vi "Call Get HW Config.vi"(8 "error in":errorcluster, 10 "Refresh Modules":bool, 11 "serverName":string) -> (0 "error out":errorcluster, 3 "HW Config":T1)   [LabVIEW 2020, in "SEECD System Explorer.lvlib"]
uses:
  SEECD System Explorer.lvlib
  Type Defs/Host - HW Config.ctl
  Type Defs/Host - Master.ctl
  Type Defs/Host - Slave.ctl
  Type Defs/IOV Container Contents.ctl
  Type Defs/Host - Module.ctl
  Type Defs/Host - Local Chassis.ctl
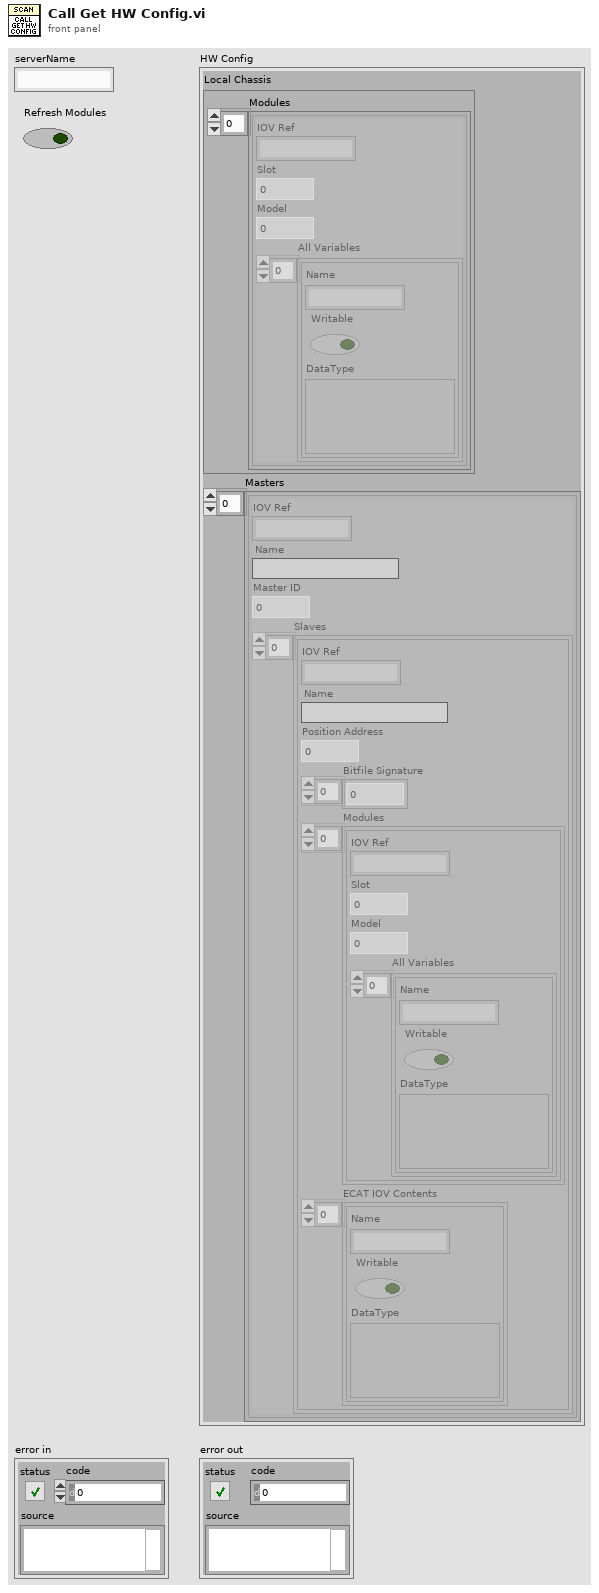
[diagram p1: front panel]
types:
  T1 = typedef "SEECD System Explorer.lvlib/Host - HW Config.ctl" = cluster{"Local Chassis":T2, "Masters":T5[]}
  T2 = typedef "SEECD System Explorer.lvlib/Host - Local Chassis.ctl" = cluster{"Modules":T3[]}
  T3 = typedef "SEECD System Explorer.lvlib/Host - Module.ctl" = cluster{"IOV Ref":string, "Slot":u32, "Model":u32, "All Variables":T4[]}
  T4 = typedef "SEECD System Explorer.lvlib/IOV Container Contents.ctl" = cluster{"Name":string, "Writable":bool, "DataType":variant}
  T5 = typedef "SEECD System Explorer.lvlib/Host - Master.ctl" = cluster{"IOV Ref":string, "Name":string, "Master ID":u32, "Slaves":T6[]}
  T6 = typedef "SEECD System Explorer.lvlib/Host - Slave.ctl" = cluster{"IOV Ref":string, "Name":string, "Position Address":u16, "Bitfile Signature":u8[], "Modules":T3[], "ECAT IOV Contents":T4[]}
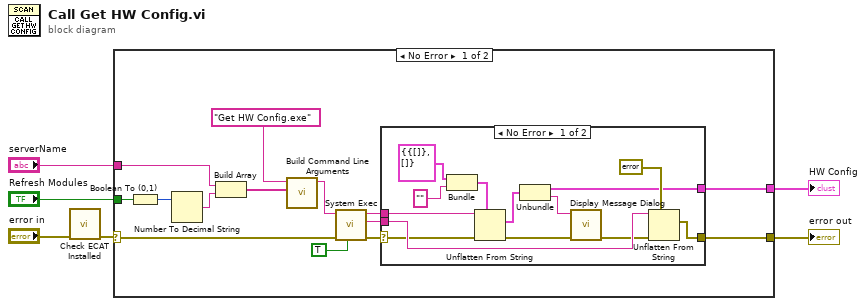
[diagram p0: block diagram]
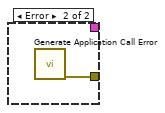
[diagram p2: hidden frame]
diagram:
  n1 = call "Check ECAT Installed.vi"("error in"="error in") -> ("error out"=w1:errorcluster)  [unwired: 10 in]
  n2 = case shown="No Error" w1 {
    selector: w1 -> [w20 w35]
    tunnel: [w7 w35] -> w6
    tunnel: "serverName" -> [w13 _]
    tunnel: [w19 _] -> w3
    tunnel: "Refresh Modules" -> [w10 _]
    frame No Error {
      n3 = Boolean To (0,1)(Boolean=w10) -> (0, 1=w9:i16)
      n4 = Number To Decimal String(number=w9) -> (decimal integer string=w8:string)  [unwired: 1 in]
      n5 = Build Array(w13, w8) -> (w12:string[])
      n6 = call "Build Command Line Arguments.vi"("Arguments"=w12, "Executable File Name"="Get HW Config.exe" ("name or relative path")) -> ("Command Line"=w11:string)  [unwired: 9 in]
      n7 = call <vilib>:"System Exec.vi"("run minimized? (F)"=TRUE, "error in (no error)"=w20, "command line"=w11) -> ("error out"=w18:errorcluster, "standard error"=w16:string, "standard output"=w17:string)  [unwired: 5 in, 1 out]
      n8 = case shown="No Error" w18 {
        selector: w18 -> [w30 _]
        tunnel: [w22 _] -> w19
        tunnel: [w32 w34] -> w7
        tunnel: w17 -> [w29 _]
        tunnel: w16 -> [w31 _]
        frame No Error {
          n9 = Bundle("HW Config"=T1 {"Local Chassis"={"Modules"=[]}, "Masters"=[]}, "") -> (w28:cluster{"HW Config":T1, string})  [unwired: 1 in]
          n10 = Unflatten From String(type=w28, binary string=w29, error in (no error)=w30) -> (value=w23:cluster{"HW Config":T1, string}, error out=w25:errorcluster)  [unwired: 2 in, 1 out]
          n11 = Unbundle(w23) -> ("HW Config"=w22:T1, w21:string)
          n12 = call "Display Message Dialog.vi"("error in"=w25, "Message to display"=w21) -> ("error out"=w24:errorcluster)  [unwired: 9 in]
          n13 = Unflatten From String(type=errorcluster {"status"=FALSE, "code"=0, "source"=""} ("error in (no error)"), binary string=w31, error in (no error)=w24) -> (value=w32:errorcluster)  [unwired: 2 in, 2 out]
        }
        frame Error {
          n14 = call "Generate Application Call Error.vi"() -> ("error out"=w34:errorcluster)  [unwired: 11 in]
        }
      }
    }
    frame Error {
    }
  }
  "HW Config" <- w3
  "error out" <- w6
